vi "Measurement UI.vi"() -> ()   [LabVIEW 2021, in "Multi-Channel Output Voltage Accuracy_PMIC.lvlib"]
uses:
  Multi-Channel Output Voltage Accuracy_PMIC.lvlib
panel:
  in  "MeasGraphs":T1(tab)
  out "LoadVoltageGraph":waveform(dbl)[](graph) caption="AC"
  in  "Load senses":i32[](array[ring]) items=["Local"=1008, "Remote"=1009]
  out "Maximum Vout(V)":dbl[](array[numeric])
  out "Minimum Vout(V)":dbl[](array[numeric])
  out "Average Vout Accuracy(V)":dbl[](array[numeric])
  out "Average Vout Deviation(%)":dbl[](array[numeric])
  out "Average Measured Vout(V)":dbl[](array[numeric])
  out "Output channel alias":string[](array[string])
  in  "Output channel alias":string[](array[string])
  in  "Load voltage limit ranges":dbl[](array[numeric])
  out "Load voltages":dbl[](array[numeric])
  in  "Nominal Vout":dbl[](array[numeric])
  in  "Load current levels":dbl[](array[numeric])
  in  "Load resource names":string[](array[string])
  in  "Source resource name":string caption="RESOURCE NAME"
  out "dt":dbl[](array[numeric])
  out "MeasTable":string[][](table)
  in  "Source sense":i32(ring)=1009 caption="SENSE" items=["Local"=1008, "Remote"=1009]
  out "Status":string
  in  "Load configuration parameters":T2(array[cluster]) {"Load sense" items=["Local"=1008, "Remote"=1009]; "Nominal Vout" format="%#_6pV"; "Load voltage limit range" format="%#_6pV"; "Load current level" format="%#_6pA"}
  in  "PPSResourceName":refnum<k15> caption="RESOURCE NAME"
  in  "DUT setup time":dbl=1.0 caption="DUT SETUP TIME" format="%#_6ps"
  in  "Measurement time":dbl=0.005 caption="MEASUREMENT TIME" format="%#_6ps"
  in  "Aperture time":dbl=0.005 caption="APERTURE TIME" format="%#_6ps"
  in  "Source voltage level":dbl=6.0 caption="VOLTAGE LEVEL" format="%#_6pV"
  in  "Source current limit":dbl=25.0 caption="CURRENT LIMIT" format="%#_6pA"
  in  "Load configuration":string="Load configuration"
  in  "Source configuration":string="Source configuration"
  in  "Measurement settings":string="Measurement settings"
  in  "Mode of operation":T3(ring)=enum."Perform measurement" caption="MODE OF OPERATION"
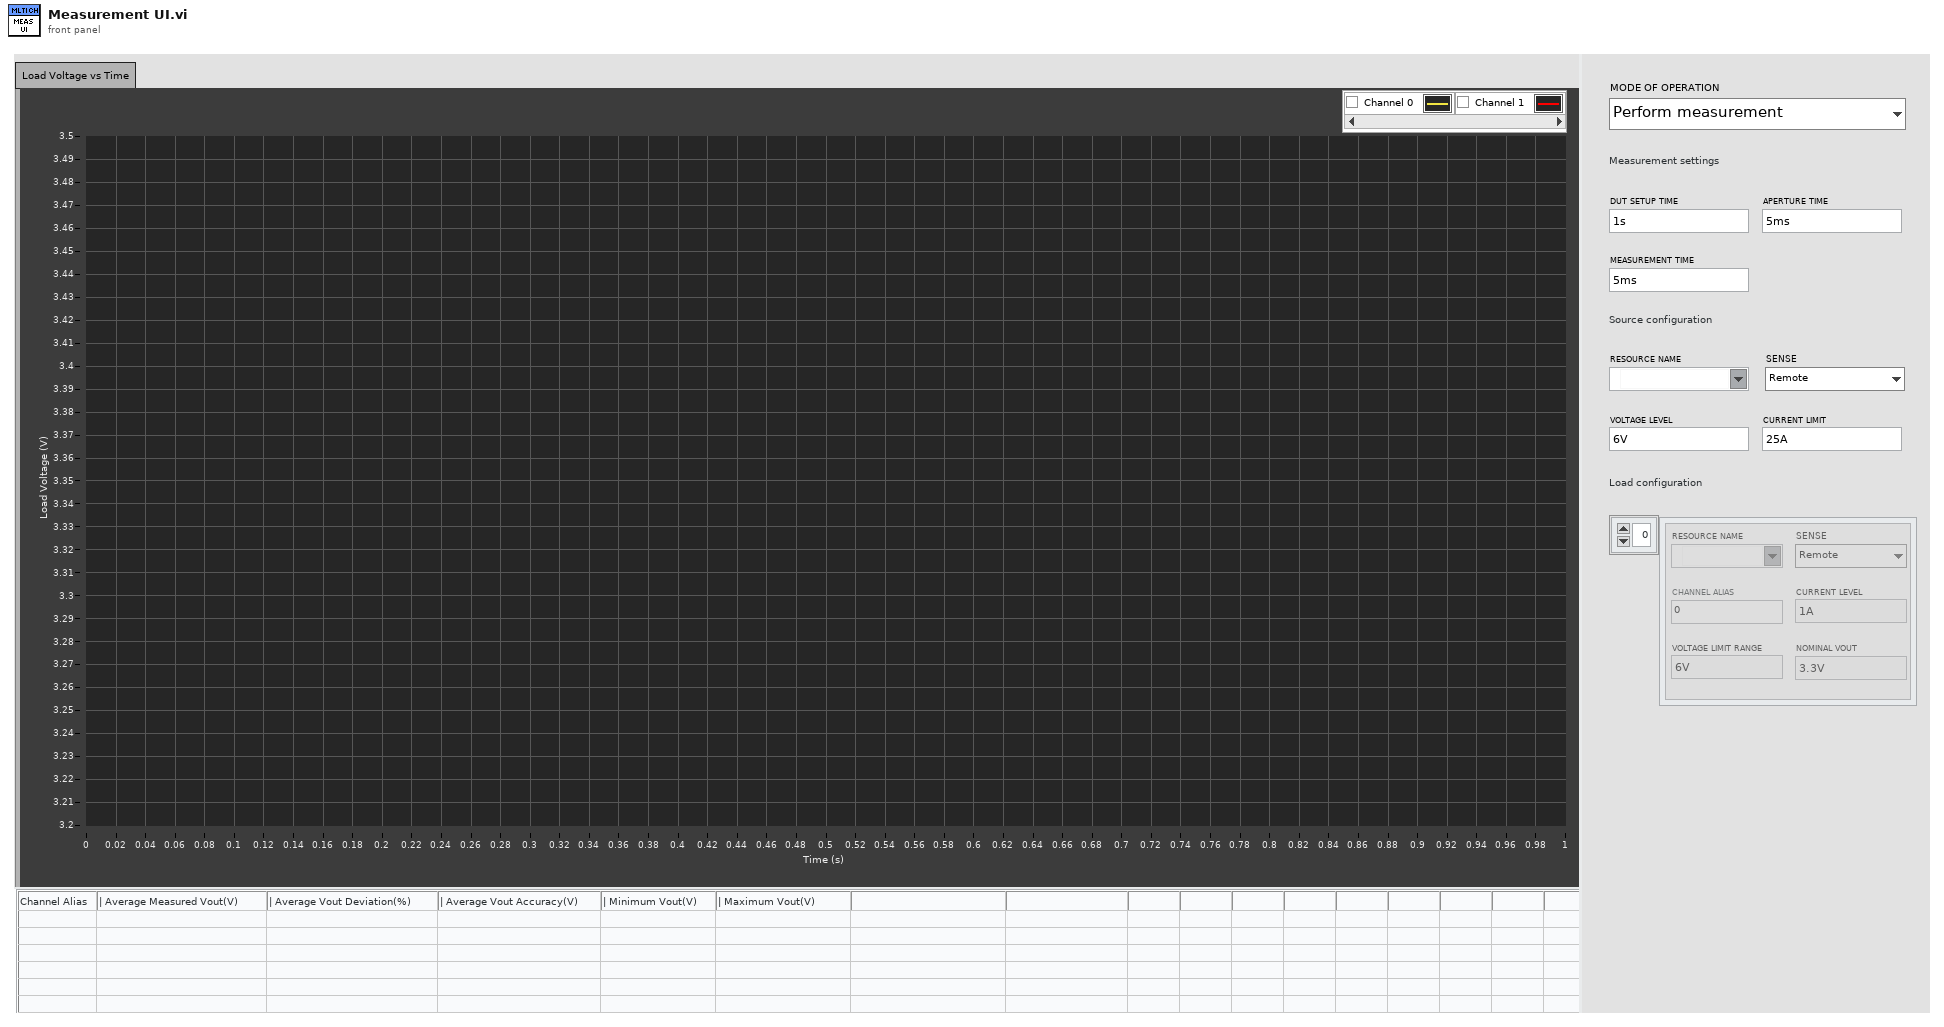
[diagram p1: front panel]
types:
  T1 = enum32{"Load Voltage vs Time", "Hidden Controls"}
  T2 = cluster{"ELOADResourceName":refnum<k15>, "Load current level":dbl, "Load voltage limit range":dbl, "Input channel":string, "Nominal Vout":dbl, "Load sense":i32}[]
  T3 = enum32{"Power on the DUT", "Perform measurement", "Power off the DUT"}
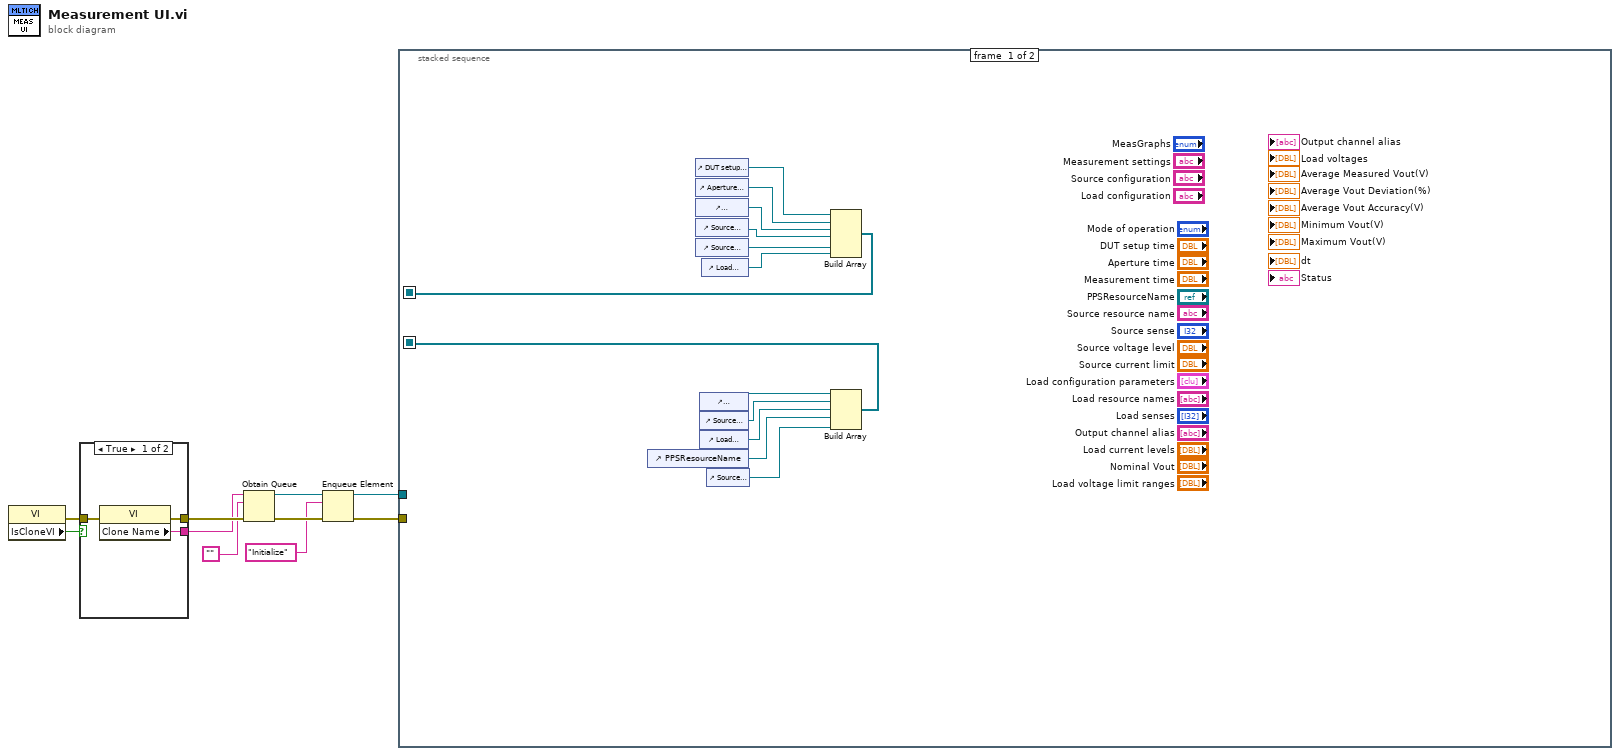
[diagram p0: block diagram]
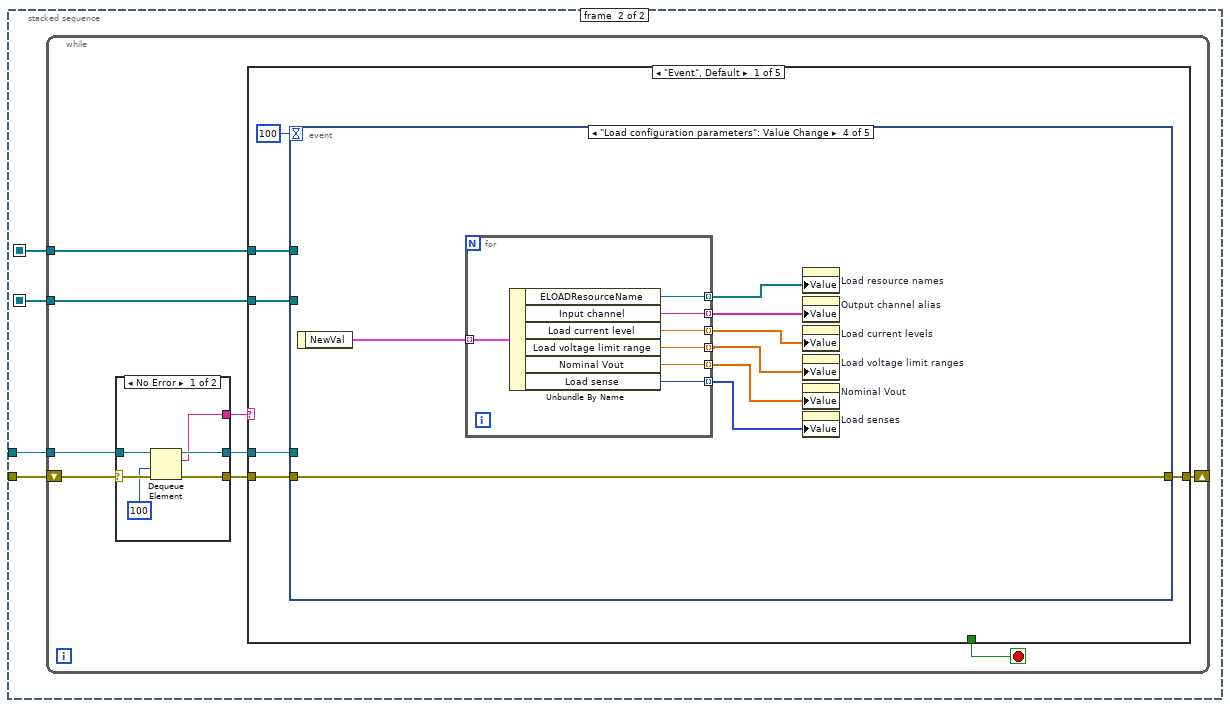
[diagram p2: hidden frame]
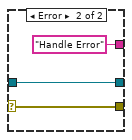
[diagram p3: hidden frame]
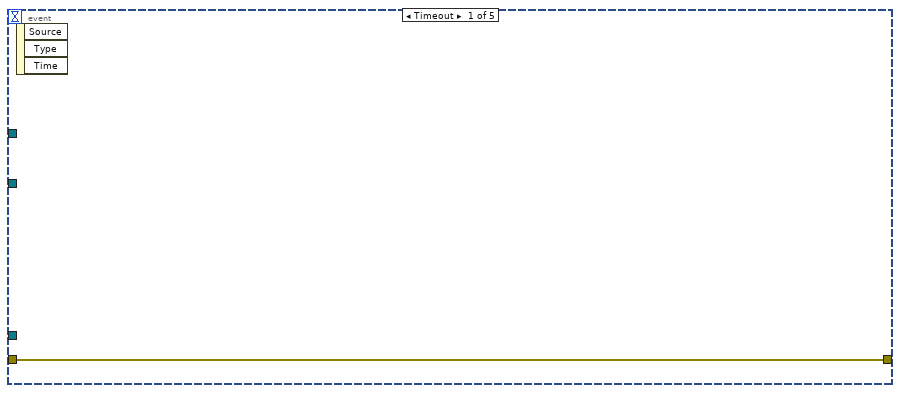
[diagram p4: hidden frame]
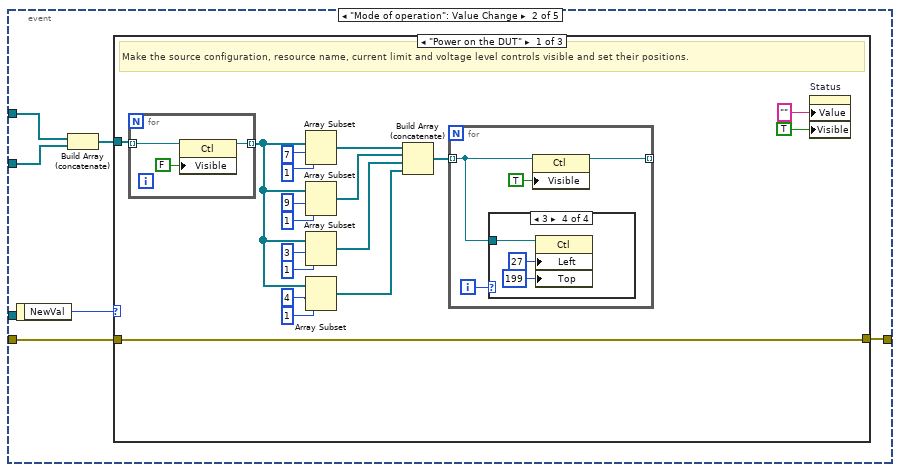
[diagram p5: hidden frame]
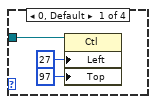
[diagram p6: hidden frame]
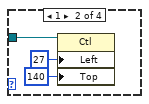
[diagram p7: hidden frame]
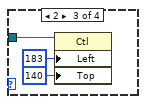
[diagram p8: hidden frame]
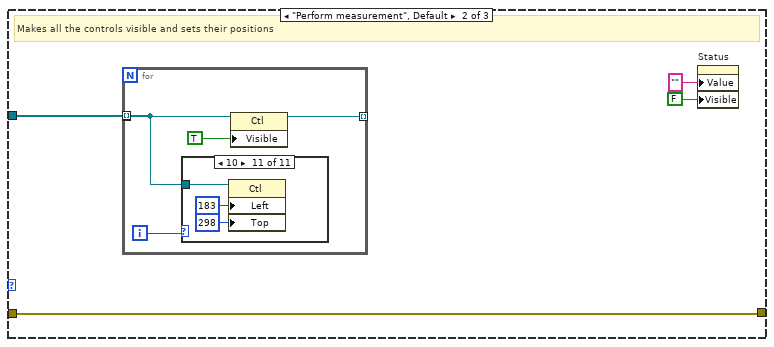
[diagram p9: hidden frame]
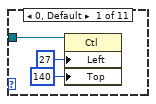
[diagram p10: hidden frame]
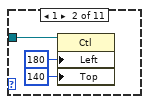
[diagram p11: hidden frame]
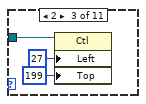
[diagram p12: hidden frame]
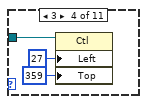
[diagram p13: hidden frame]
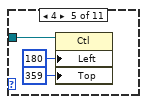
[diagram p14: hidden frame]
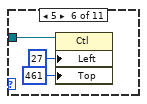
[diagram p15: hidden frame]
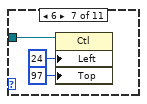
[diagram p16: hidden frame]
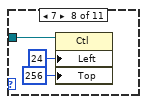
[diagram p17: hidden frame]
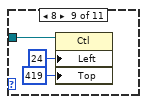
[diagram p18: hidden frame]
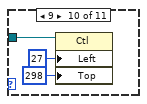
[diagram p19: hidden frame]
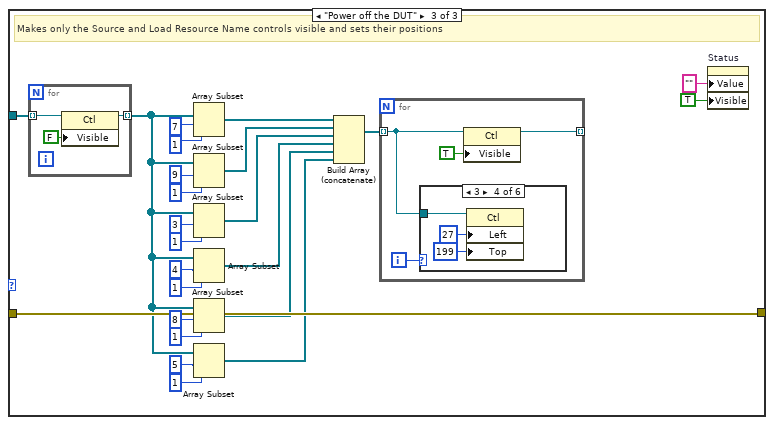
[diagram p20: hidden frame]
diagram:
  n1 = property class="VI"() -> (error out=w1:errorcluster, "IsCloneVI"=w2:bool)  [unwired: 2 in, 1 out]
  n2 = case shown="True" w2 {
    tunnel: [w13 w16] -> w10
    tunnel: [w12 w15] -> w9
    tunnel: w1 -> [w11 w14]
    frame True {
      n3 = property class="VI"(error in=w11) -> (error out=w13:errorcluster, "Clone Name"=w12:string)  [unwired: 1 in, 1 out]
    }
    frame False {
      n4 = property class="VI"(error in=w14) -> (error out=w16:errorcluster, "Name"=w15:string)  [unwired: 1 in, 1 out]
    }
  }
  n5 = Obtain Queue(name (unnamed)=w9, element data type="", error in (no error)=w10) -> (queue out=w6:refnum<queue>, error out=w8:errorcluster)  [unwired: 2 in, 1 out]
  n6 = Enqueue Element(queue=w6, element="Initialize", error in (no error)=w8) -> (queue out=w5:refnum<queue>, error out=w7:errorcluster)  [unwired: 1 in, 1 out]
  n7 = stacked-sequence {
    seq-local: [w19 _] -> [_ w31]
    seq-local: [w18 _] -> [_ w30]
    tunnel: w7 -> [_ w33]
    tunnel: w5 -> [_ w32]
    frame #0 {
      n8 = control-ref of="PPSResourceName"() -> (w20:refnum<vi>)
      n9 = control-ref of="DUT setup time"() -> (w29:refnum<vi>)
      n10 = control-ref of="Aperture time"() -> (w28:refnum<vi>)
      n11 = control-ref of="Measurement time"() -> (w27:refnum<vi>)
      n12 = control-ref of="Source voltage level"() -> (w26:refnum<vi>)
      n13 = control-ref of="Source current limit"() -> (w25:refnum<vi>)
      n14 = control-ref of="Measurement settings"() -> (w23:refnum<vi>)
      n15 = control-ref of="Source configuration"() -> (w22:refnum<vi>)
      n16 = control-ref of="Load configuration"() -> (w21:refnum<vi>)
      n17 = control-ref of="Load configuration parameters"() -> (w24:refnum<vi>)
      n18 = control-ref of="Source sense"() -> (w17:refnum<vi>)
      n19 = Build Array(w29, w28, w27, w26, w25, w24) -> (w19:refnum<vi>[])
      n20 = Build Array(w23, w22, w21, w20, w17) -> (w18:refnum<vi>[])
    }
    frame #1 {
      n21 = while {
        shift-right: [w37] -> _
        shift-left: w33 -> [w42]
        tunnel: w32 -> [w40]
        tunnel: w31 -> [w35]
        tunnel: w30 -> [w34]
        stop <- w36 stop-if-true
        n22 = case shown="No Error" w42 {
          selector: w42 -> [w48 w51]
          tunnel: [w47 w51] -> w41
          tunnel: w40 -> [w46 w50]
          tunnel: [w45 w50] -> w39
          tunnel: [w44 "Handle Error"] -> w38
          frame No Error {
            n23 = Dequeue Element(queue=w46, timeout in ms (-1)=100, error in (no error)=w48) -> (queue out=w45:refnum<queue>, element=w44:string, error out=w47:errorcluster)  [unwired: 1 out]
          }
          frame Error {
          }
        }
        n24 = case shown="\"Event\", Default" w38 {
          tunnel: w41 -> [w56 w214 w222 w263 w264]
          tunnel: w39 -> [w54 _ _ w261 _]
          tunnel: [w57 w214 w222 w258 w264] -> w37
          tunnel: [_ FALSE _ TRUE _] -> w36
          tunnel: w35 -> [w53 _ _ _ _]
          tunnel: w34 -> [w52 _ _ _ _]
          frame "Event", Default {
            n25 = event shown="[3] \"Load configuration parameters\": Value Change" {
              selector: _ -> [_ _ _ _ _]
              dyn-events: _ -> [_ _ _ _ _]
              timeout: 100 -> [_ _ _ _ _]
              tunnel: [w58 w59 _ w194 w210] -> w57
              tunnel: w56 -> [w58 w60 _ w194 w211]
              tunnel: w54 -> [_ _ _ _ w209]
              tunnel: w53 -> [_ w63 _ _ _]
              tunnel: w52 -> [_ w62 _ _ _]
              event Timeout {
                n26 = event-data() -> ()  [unwired: 1 in, 3 out]
              }
              event "Mode of operation": Value Change {
                n27 = event-data() -> ("NewVal"=w64:T3)  [unwired: 1 in]
                n28 = Build Array (concatenate)(w63, w62) -> (w61:refnum<vi>[])
                n29 = case shown="\"Power on the DUT\"" w64 {
                  tunnel: w61 -> [w74 w103 w150]
                  tunnel: w60 -> [w65 w102 w164]
                  tunnel: [w65 w102 w164] -> w59
                  frame "Power on the DUT" {
                    # "Make the source configuration, resource name, current limit and voltage level controls visible and set their positions."
                    n30 = for {
                      tunnel: w74 -> [w85] mode=indexing
                      tunnel: [w83] -> w71 mode=indexing
                      n31 = property class="Ctl"(reference=w85, "Visible"=FALSE) -> (reference out=w83:refnum<vi>)  [unwired: 1 in, 1 out]
                    }
                    n32 = Array Subset(array=w71, index=7 ("length"), length=1 ("index")) -> (w73:refnum<vi>[])
                    n33 = Array Subset(array=w71, index=9 ("length"), length=1 ("index")) -> (w72:refnum<vi>[])
                    n34 = Array Subset(array=w71, index=3 ("length"), length=1 ("index")) -> (w70:refnum<vi>[])
                    n35 = Array Subset(array=w71, index=4 ("length"), length=1 ("index")) -> (w68:refnum<vi>[])
                    n36 = Build Array (concatenate)(w73, w72, w70, w68) -> (w69:refnum<vi>[])
                    n37 = for {
                      tunnel: [w88] -> _ mode=indexing
                      tunnel: w69 -> [w86] mode=indexing
                      i -> [w87]
                      n38 = case shown="3" w87 {
                        tunnel: w86 -> [w92 w95 w98 w101]
                        frame 0, Default {
                          n39 = property class="Ctl"(reference=w92, "Left"=27 ("Position:Left"), "Top"=97 ("Position:Top")) -> ()  [unwired: 1 in, 2 out]
                        }
                        frame 1 {
                          n40 = property class="Ctl"(reference=w95, "Left"=27 ("Position:Left"), "Top"=140 ("Position:Top")) -> ()  [unwired: 1 in, 2 out]
                        }
                        frame 2 {
                          n41 = property class="Ctl"(reference=w98, "Left"=183 ("Position:Left"), "Top"=140 ("Position:Top")) -> ()  [unwired: 1 in, 2 out]
                        }
                        frame 3 {
                          n42 = property class="Ctl"(reference=w101, "Left"=27 ("Position:Left"), "Top"=199 ("Position:Top")) -> ()  [unwired: 1 in, 2 out]
                        }
                      }
                      n43 = property class="Ctl"(reference=w86, "Visible"=TRUE) -> (reference out=w88:refnum<vi>)  [unwired: 1 in, 1 out]
                    }
                    n44 = property on="Status" class="Str"("Value"="" ("Status"), "Visible"=TRUE) -> ()  [unwired: 2 in, 2 out]
                  }
                  frame "Perform measurement", Default {
                    # "Makes all the controls visible and sets their positions"
                    n45 = for {
                      tunnel: [w106] -> _ mode=indexing
                      tunnel: [w108] -> _ mode=indexing
                      tunnel: w103 -> [w106] mode=indexing
                      i -> [w107]
                      n46 = case shown="10" w107 {
                        tunnel: w106 -> [w112 w115 w118 w121 w124 w127 w130 w133 w136 w139 w140]
                        frame 0, Default {
                          n47 = property class="Ctl"(reference=w112, "Left"=27 ("Position:Left"), "Top"=140 ("Position:Top")) -> ()  [unwired: 1 in, 2 out]
                        }
                        frame 1 {
                          n48 = property class="Ctl"(reference=w115, "Left"=180 ("Position:Left"), "Top"=140 ("Position:Top")) -> ()  [unwired: 1 in, 2 out]
                        }
                        frame 2 {
                          n49 = property class="Ctl"(reference=w118, "Left"=27 ("Position:Left"), "Top"=199 ("Position:Top")) -> ()  [unwired: 1 in, 2 out]
                        }
                        frame 3 {
                          n50 = property class="Ctl"(reference=w121, "Left"=27 ("Position:Left"), "Top"=359 ("Position:Top")) -> ()  [unwired: 1 in, 2 out]
                        }
                        frame 4 {
                          n51 = property class="Ctl"(reference=w124, "Left"=180 ("Position:Left"), "Top"=359 ("Position:Top")) -> ()  [unwired: 1 in, 2 out]
                        }
                        frame 5 {
                          n52 = property class="Ctl"(reference=w127, "Left"=27 ("Position:Left"), "Top"=461 ("Position:Top")) -> ()  [unwired: 1 in, 2 out]
                        }
                        frame 6 {
                          n53 = property class="Ctl"(reference=w130, "Left"=24 ("Position:Left"), "Top"=97 ("Position:Top")) -> ()  [unwired: 1 in, 2 out]
                        }
                        frame 7 {
                          n54 = property class="Ctl"(reference=w133, "Left"=24 ("Position:Left"), "Top"=256 ("Position:Top")) -> ()  [unwired: 1 in, 2 out]
                        }
                        frame 8 {
                          n55 = property class="Ctl"(reference=w136, "Left"=24 ("Position:Left"), "Top"=419 ("Position:Top")) -> ()  [unwired: 1 in, 2 out]
                        }
                        frame 9 {
                          n56 = property class="Ctl"(reference=w139, "Left"=27 ("Position:Left"), "Top"=298 ("Position:Top")) -> ()  [unwired: 1 in, 2 out]
                        }
                        frame 10 {
                          n57 = property class="Ctl"(reference=w140, "Left"=183 ("Position:Left"), "Top"=298 ("Position:Top")) -> ()  [unwired: 1 in, 2 out]
                        }
                      }
                      n58 = property class="Ctl"(reference=w106, "Visible"=TRUE) -> (reference out=w108:refnum<vi>)  [unwired: 1 in, 1 out]
                    }
                    n59 = property on="Status" class="Str"("Value"="" ("Status"), "Visible"=FALSE) -> ()  [unwired: 2 in, 2 out]
                  }
                  frame "Power off the DUT" {
                    # "Makes only the Source and Load Resource Name controls visible and sets their positions"
                    n60 = for {
                      tunnel: w150 -> [w168] mode=indexing
                      tunnel: [w167] -> w145 mode=indexing
                      n61 = property class="Ctl"(reference=w168, "Visible"=FALSE) -> (reference out=w167:refnum<vi>)  [unwired: 1 in, 1 out]
                    }
                    n62 = Array Subset(array=w145, index=7 ("length"), length=1 ("index")) -> (w155:refnum<vi>[])
                    n63 = Array Subset(array=w145, index=9 ("length"), length=1 ("index")) -> (w154:refnum<vi>[])
                    n64 = Array Subset(array=w145, index=3 ("length"), length=1 ("index")) -> (w153:refnum<vi>[])
                    n65 = Array Subset(array=w145, index=4 ("length"), length=1 ("index")) -> (w151:refnum<vi>[])
                    n66 = Array Subset(array=w145, index=8 ("length"), length=1 ("index")) -> (w144:refnum<vi>[])
                    n67 = Array Subset(array=w145, index=5 ("length"), length=1 ("index")) -> (w143:refnum<vi>[])
                    n68 = Build Array (concatenate)(w155, w154, w153, w151, w144, w143) -> (w152:refnum<vi>[])
                    n69 = for {
                      tunnel: [w172] -> _ mode=indexing
                      tunnel: w152 -> [w170] mode=indexing
                      i -> [w171]
                      n70 = case shown="3" w171 {
                        tunnel: w170 -> [w176 w179 w182 w185 w186 w189]
                        frame 0, Default {
                          n71 = property class="Ctl"(reference=w176, "Left"=24 ("Position:Left"), "Top"=97 ("Position:Top")) -> ()  [unwired: 1 in, 2 out]
                        }
                        frame 1 {
                          n72 = property class="Ctl"(reference=w179, "Left"=27 ("Position:Left"), "Top"=140 ("Position:Top")) -> ()  [unwired: 1 in, 2 out]
                        }
                        frame 2 {
                          n73 = property class="Ctl"(reference=w182, "Left"=183 ("Position:Left"), "Top"=140 ("Position:Top")) -> ()  [unwired: 1 in, 2 out]
                        }
                        frame 3 {
                          n74 = property class="Ctl"(reference=w185, "Left"=27 ("Position:Left"), "Top"=199 ("Position:Top")) -> ()  [unwired: 1 in, 2 out]
                        }
                        frame 4 {
                          n75 = property class="Ctl"(reference=w186, "Left"=27 ("Position:Left"), "Top"=254 ("Position:Top")) -> ()  [unwired: 1 in, 2 out]
                        }
                        frame 5 {
                          n76 = property class="Ctl"(reference=w189, "Left"=27 ("Position:Left"), "Top"=303 ("Position:Top")) -> ()  [unwired: 1 in, 2 out]
                        }
                      }
                      n77 = property class="Ctl"(reference=w170, "Visible"=TRUE) -> (reference out=w172:refnum<vi>)  [unwired: 1 in, 1 out]
                    }
                    n78 = property on="Status" class="Str"("Value"="" ("Status"), "Visible"=TRUE) -> ()  [unwired: 2 in, 2 out]
                  }
                }
              }
              event "PPSResourceName": Value Change {
                n79 = event-data() -> ("NewVal"=w192:refnum<k15>)  [unwired: 1 in]
                n80 = property on="Source resource name" class="Str"("Value"=w192) -> ()  [unwired: 2 in, 2 out]
              }
              event "Load configuration parameters": Value Change {
                n81 = event-data() -> ("NewVal"=w200:T2)  [unwired: 1 in]
                n82 = for {
                  tunnel: w200 -> [w207] mode=indexing
                  tunnel: [w206] -> w199 mode=indexing
                  tunnel: [w205] -> w198 mode=indexing
                  tunnel: [w204] -> w195 mode=indexing
                  tunnel: [w203] -> w197 mode=indexing
                  tunnel: [w202] -> w196 mode=indexing
                  tunnel: [w201] -> w193 mode=indexing
                  n83 = Unbundle By Name(w207) -> ("ELOADResourceName"=w206:refnum<k15>, "Input channel"=w205:string, "Load current level"=w204:dbl, "Load voltage limit range"=w203:dbl, "Nominal Vout"=w202:dbl, "Load sense"=w201:i32)
                }
                n84 = property on="Load resource names" class="Arr (strict)"("Value"=w199) -> ()  [unwired: 2 in, 2 out]
                n85 = property on="Output channel alias" class="Arr (strict)"("Value"=w198) -> ()  [unwired: 2 in, 2 out]
                n86 = property on="Load current levels" class="Arr (strict)"("Value"=w195) -> ()  [unwired: 2 in, 2 out]
                n87 = property on="Load voltage limit ranges" class="Arr (strict)"("Value"=w197) -> ()  [unwired: 2 in, 2 out]
                n88 = property on="Nominal Vout" class="Arr (strict)"("Value"=w196) -> ()  [unwired: 2 in, 2 out]
                n89 = property on="Load senses" class="Arr (strict)"("Value"=w193) -> ()  [unwired: 2 in, 2 out]
              }
              event Panel Close? {
                n90 = event-data() -> ()  [unwired: 1 in, 4 out]
                n91 = Enqueue Element(queue=w209, element="Exit", error in (no error)=w211) -> (error out=w210:errorcluster)  [unwired: 1 in, 2 out]
                n92 = event-data("Discard?"=TRUE) -> ()  [unwired: 1 in, 1 out]
              }
            }
          }
          frame "Initialize" {
          }
          frame "Post UI Update" {
            # "This case will be triggered, after framework updates the User interface with result values."
            n93 = local read "Output channel alias"() -> (w220:string[])
            n94 = local read "Average Measured Vout(V)"() -> (w223:dbl[])
            n95 = local read "Average Vout Deviation(%)"() -> (w221:dbl[])
            n96 = local read "Load voltages"() -> (w228:dbl[])
            n97 = local read "Average Vout Accuracy(V)"() -> (w217:dbl[])
            n98 = for {
              tunnel: w220 -> [w231] mode=indexing
              tunnel: [w231] -> w219 mode=indexing
              i -> [w230]
              n99 = property on="LoadVoltageGraph" class="WFGraph (strict)"("Active Plot"=w230, "Plot.Plot Name"=w231) -> ()  [unwired: 2 in, 2 out]
            }
            n100 = local read "Maximum Vout(V)"() -> (w216:dbl[])
            n101 = local read "Minimum Vout(V)"() -> (w218:dbl[])
            n102 = local read "dt"() -> (w225:dbl[])
            n103 = Array Size(array=w228) -> (size(s)=w227:i32)
            n104 = Array Size(array=w225) -> (size(s)=w215:i32)
            n105 = Divide(x=w227, y=w215) -> (x/y=w226:dbl)
            n106 = for {
              N: w215 -> [_]
              tunnel: [w256] -> w229 mode=indexing
              tunnel: w226 -> [w254]
              shift-right: [w252] -> _
              shift-left: w228 -> [w255]
              tunnel: w225 -> [w250] mode=indexing
              n107 = Delete From Array(array=w255, length=w254, index=0) -> (deleted portion=w253:dbl[], array with subset deleted=w252:dbl[])
              n108 = Bundle By Name("dt"=w250, "Y"=w253) -> (w256:waveform(dbl))  [unwired: 1 in]
            }
            "LoadVoltageGraph" <- w229
            n109 = for {
              N: w215 -> [_]
              tunnel: w217 -> [w239] mode=indexing
              tunnel: w223 -> [w241] mode=indexing
              tunnel: [w247] -> w224 mode=indexing
              tunnel: w219 -> [w246] mode=indexing
              tunnel: w221 -> [w240] mode=indexing
              tunnel: w218 -> [w238] mode=indexing
              tunnel: w216 -> [w237] mode=indexing
              w232 = "|" ("initial string")
              n110 = Format Into String(format string="%0.9f" ("initial string"), w241) -> (resulting string=w248:string)  [unwired: 2 in, 1 out]
              n111 = Format Into String(format string="%0.9f" ("initial string"), initial string=w232, w240) -> (resulting string=w236:string)  [unwired: 1 in, 1 out]
              n112 = Format Into String(format string="%0.9f" ("initial string"), initial string=w232, w239) -> (resulting string=w235:string)  [unwired: 1 in, 1 out]
              n113 = Format Into String(format string="%0.9f" ("initial string"), initial string=w232, w238) -> (resulting string=w234:string)  [unwired: 1 in, 1 out]
              n114 = Format Into String(format string="%0.9f" ("initial string"), initial string=w232, w237) -> (resulting string=w233:string)  [unwired: 1 in, 1 out]
              n115 = Build Array(w246, w248, w236, w235, w234, w233) -> (w247:string[])
            }
            "MeasTable" <- w224
          }
          frame "Exit" {
            # "This case is triggered to close the User Interface from framework"
            n116 = Flush Queue(queue=w261, error in (no error)=w263) -> (queue out=w260:refnum<queue>, error out=w259:errorcluster)  [unwired: 1 out]
            n117 = Release Queue(queue=w260, force destroy? (F)=TRUE, error in (no error)=w259) -> (error out=w258:errorcluster)  [unwired: 2 out]
          }
          frame "Handle Error" {
          }
        }
      }
    }
  }
